vi "Heartbeat.vi"() -> ()   [LabVIEW 2026]
doc: "Degenerate single-state machine: a state that transitions to itself, exercising the wrap-around path."
panel:
  out "History":enum16{"Only"}[](array[ring])
  out "Cycles":i32
  out "Final Tick":i32
  out "Final State":enum16{"Only"}(ring)
  in  "Max Cycles":i32=3
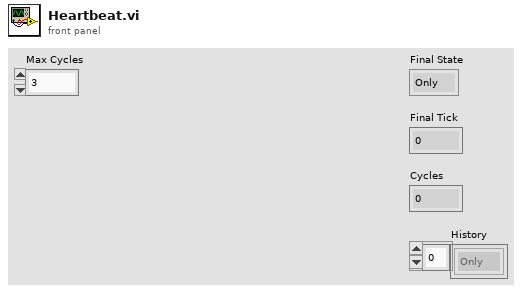
[diagram p1: front panel]
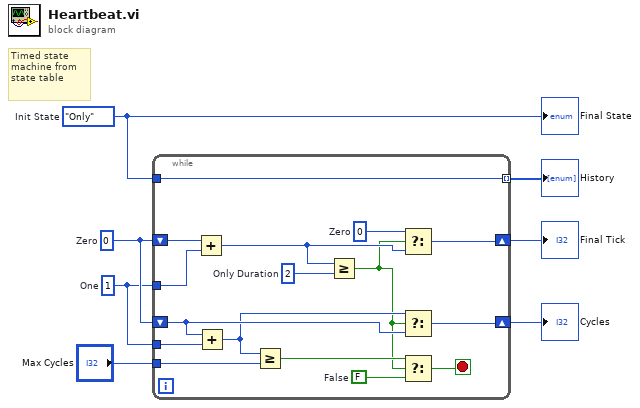
[diagram p0: block diagram]
diagram:
  w5 = 1  # One
  w6 = 0  # Zero
  w4 = enum16{"Only"}."Only"  # Init State
  # "Timed state machine from state table"
  n1 = while {
    tunnel: "Max Cycles" -> [w12]
    tunnel: w4 -> [w23]
    tunnel: [w23] -> w1 mode=indexing
    shift-right: [w17] -> w3
    shift-left: w6 -> [w22]
    shift-right: [w14] -> w2
    shift-left: w6 -> [w15]
    tunnel: w5 -> [w21]
    tunnel: w5 -> [w16]
    stop <- w8 stop-if-true
    w9 = FALSE  # False
    w19 = 0  # Zero
    w20 = 2  # Only Duration
    n2 = Add(x=w22, y=w21) -> (x+y=w18:i32)
    n3 = Add(x=w15, y=w16) -> (x+y=w13:i32)
    n4 = Greater Or Equal?(x=w13, y=w12) -> (x >= y?=w11:bool)
    n5 = Greater Or Equal?(x=w18, y=w20) -> (x >= y?=w10:bool)
    n6 = Select(t=w19, s=w10, f=w18) -> (s? t:f=w17:i32)
    n7 = Select(t=w13, s=w10, f=w15) -> (s? t:f=w14:i32)
    n8 = Select(t=w11, s=w10, f=w9) -> (s? t:f=w8:bool)
  }
  "Final Tick" <- w3
  "Cycles" <- w2
  "History" <- w1
  "Final State" <- w4
